vi "BIN-write.vi"(8 "error in":errorcluster, 10 "Data in":T2, 11 "refnum in":refnum<file>) -> (0 "error out":errorcluster, 2 "path":path, 3 "TimeRange":T1)   [LabVIEW 2020, in "Sgraph_lib_V1.lvlib" / "DBAL-BIN.lvclass"]
doc: "Write to a Binary historian file"
uses:
  DBAL-BIN.lvclass
  controls/DBAL_PAQ_TimeRange.ctl
  controls/BIN/BINdata.ctl
  DBAL.lvclass
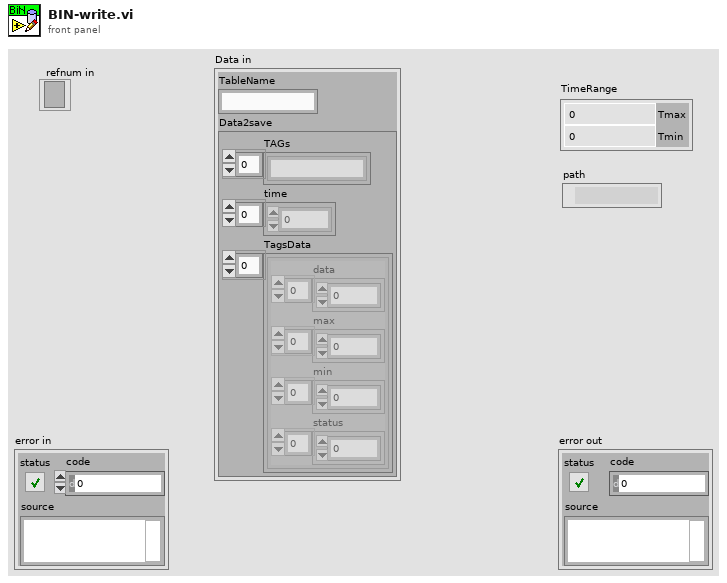
[diagram p1: front panel]
types:
  T1 = typedef "Sgraph_lib_V1.lvlib/DBAL.lvclass/DBAL_PAQ_TimeRange.ctl" = cluster{"Tmax":dbl, "Tmin":dbl}
  T2 = cluster{"TableName":string, "Data2save":cluster{"TAGs":string[], "time":dbl[], "TagsData":cluster{"data":dbl[], "max":dbl[], "min":dbl[], "status":u32[]}[]}}
  T3 = enum16{"big-endian, network order", "native, host order", "little-endian"}
  T4 = typedef "Sgraph_lib_V1.lvlib/DBAL-BIN.lvclass/BINdata.ctl" = cluster{"time":dbl[], "TagsData":cluster{"data":dbl[], "max":dbl[], "min":dbl[], "status":u32[]}[]}
  T5 = cluster{"TAGs":string[], "time":dbl[], "TagsData":cluster{"data":dbl[], "max":dbl[], "min":dbl[], "status":u32[]}[]}
  T6 = cluster{"data":dbl[], "max":dbl[], "min":dbl[], "status":u32[]}[]
  T7 = cluster{"data":dbl[], "max":dbl[], "min":dbl[], "status":u32[]}
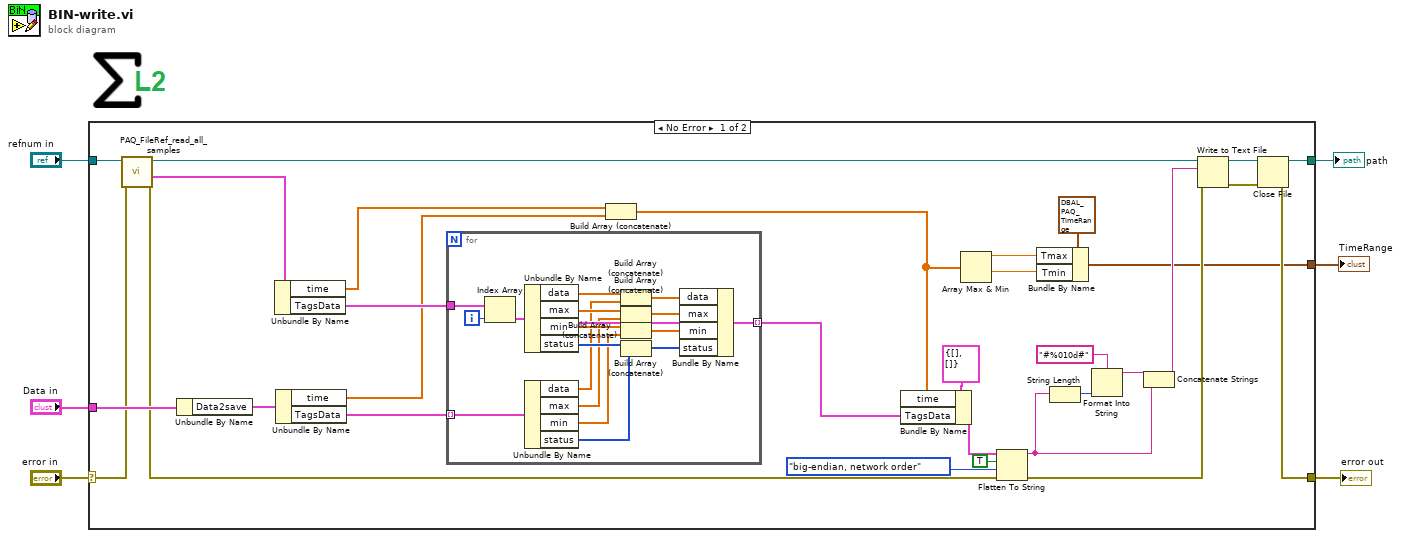
[diagram p0: block diagram]
diagram:
  n1 = case shown="No Error" "error in" {
    selector: "error in" -> [w15 w55]
    tunnel: [w37 w55] -> w5
    tunnel: "refnum in" -> [w24 _]
    tunnel: "Data in" -> [w19 _]
    tunnel: [w9 _] -> w2
    tunnel: [w8 _] -> w1
    frame No Error {
      n2 = call "PAQ_FileRef_read_all_samples.vi"("error in (no error)"=w15, "refnum in"=w24) -> ("error out"=w14:errorcluster, "data"=w20:T4, "refnum out"=w23:refnum<file>)  [unwired: 6 in, 1 out]
      n3 = Unbundle By Name(w19) -> ("Data2save"=w18:T5)
      n4 = Unbundle By Name(w20) -> ("time"=w17:dbl[], "TagsData"=w22:T6)
      n5 = Unbundle By Name(w18) -> ("time"=w16:dbl[], "TagsData"=w21:T6)
      n6 = for {
        tunnel: w21 -> [w52] mode=indexing
        tunnel: w22 -> [w54]
        tunnel: [w50] -> w13 mode=indexing
        i -> [w53]
        n7 = Index Array(array=w54, index=w53) -> (element=w51:T7)
        n8 = Unbundle By Name(w51) -> ("data"=w45:dbl[], "max"=w44:dbl[], "min"=w43:dbl[], "status"=w42:u32[])
        n9 = Unbundle By Name(w52) -> ("data"=w41:dbl[], "max"=w40:dbl[], "min"=w39:dbl[], "status"=w38:u32[])
        n10 = Build Array (concatenate)(w45, w41) -> (w47:dbl[])
        n11 = Build Array (concatenate)(w44, w40) -> (w48:dbl[])
        n12 = Build Array (concatenate)(w43, w39) -> (w49:dbl[])
        n13 = Build Array (concatenate)(w42, w38) -> (w46:u32[])
        n14 = Bundle By Name(cluster=w51, "data"=w47, "max"=w48, "min"=w49, "status"=w46) -> (w50:T7)
      }
      n15 = Build Array (concatenate)(w17, w16) -> (w12:dbl[])
      n16 = Bundle By Name(cluster=T4 {"time"=[], "TagsData"=[]} ("BinHistData"), "time"=w12, "TagsData"=w13) -> (w26:T4)
      n17 = Array Max & Min(array=w12) -> (max value=w11:dbl, min value=w10:dbl)  [unwired: 2 out]
      n18 = Flatten To String(anything=w26, prepend array or string size? (T)=TRUE, byte order (0:big-endian, network order)=T3."big-endian, network order", error in (no error)=w14) -> (data string=w25:string, error out=w29:errorcluster)  [unwired: 1 out]
      n19 = Bundle By Name(cluster=T1 {"Tmax"=3704649606.308572, "Tmin"=3704644835.5583253} ("TimeRange"), "Tmax"=w11, "Tmin"=w10) -> (w9:T1)
      n20 = String Length(string=w25) -> (length=w35:i32)
      n21 = Format Into String(format string="#%010d#", w35) -> (resulting string=w33:string)  [unwired: 2 in, 1 out]
      n22 = Concatenate Strings(w33, w25) -> (w27:string)
      n23 = Write to Text File(file (use dialog)=w23, text=w27, error in=w29) -> (refnum out=w30:refnum<file>, error out=w31:errorcluster)  [unwired: 1 in, 1 out]
      n24 = Close File(refnum=w30, error in=w31) -> (path=w8:path, error out=w37:errorcluster)
    }
    frame Error {
    }
  }
  "error out" <- w5
  "TimeRange" <- w2
  "path" <- w1
